vi "abbreviations creator.vi"   [LabVIEW 2020]
uses:
  Abbreviations.vi
  Silly Billy.lvlib
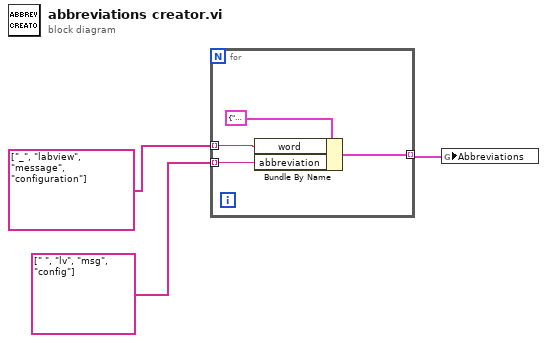
[diagram p0: block diagram]
diagram:
  n1 = for {
    tunnel: string[] ["_", "labview", "message", "configuration"] -> [w6] mode=indexing
    tunnel: string[] [" ", "lv", "msg", "config"] -> [w5] mode=indexing
    tunnel: [w4] -> w1 mode=indexing
    n2 = Bundle By Name(cluster=cluster{"word":string, "abbreviation":string} {"word"="", "abbreviation"=""}, "word"=w6, "abbreviation"=w5) -> (w4:cluster{"word":string, "abbreviation":string})
  }
  n3 = global write "Abbreviations.vi" "Abbreviations"(w1) -> ()
